vi "Send Reply.vi"(8 "错误输入（无错误）":errorcluster, 9 "Data":variant, 10 "请求":T1, 11 "Send Q":refnum<queue>) -> (0 "error out":errorcluster, 3 "Send Q":refnum<queue>)   [LabVIEW 2020, in "TCP Communication.lvlib"]
uses:
  TCP Communication.lvlib
  Requset.ctl
  Reply.ctl
  Data Type.ctl
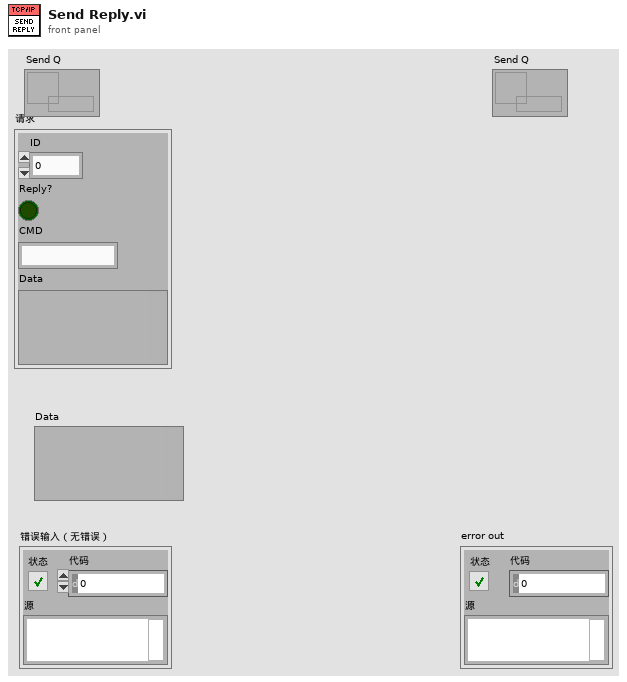
[diagram p1: front panel]
types:
  T1 = typedef "TCP Communication.lvlib/Requset.ctl" = cluster{"ID":i32, "Reply?":bool, "CMD":string, "Data":variant}
  T2 = typedef "TCP Communication.lvlib/Data Type.ctl" = enum16{"Data Stream", "Status", "Request", "Reply"}
  T3 = typedef "TCP Communication.lvlib/Reply.ctl" = cluster{"ID":i32, "CMD":string, "Data":variant}
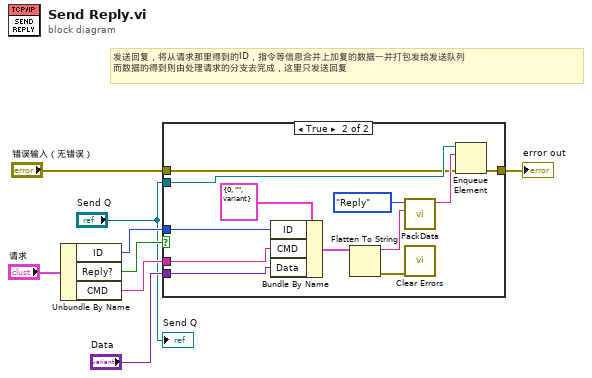
[diagram p0: block diagram]
diagram:
  # "发送回复，将从请求那里得到的ID，指令等信息合并上加复的数据一并打包发给发送队列\n而数据的得到则由处理请求的分支去完成，这里只发送回复"
  n1 = Unbundle By Name("请求") -> ("ID"=w7:i32, "Reply?"=w8:bool, "CMD"=w6:string)
  n2 = case shown="True" w8 {
    tunnel: w7 -> [_ w20]
    tunnel: w6 -> [_ w19]
    tunnel: "Send Q" -> [_ w15]
    tunnel: "Data" -> [_ w13]
    tunnel: [w9 w11] -> w3
    tunnel: "错误输入（无错误）" -> [w9 w10]
    frame False {
    }
    frame True {
      n3 = Bundle By Name(cluster=T3 {"ID"=0, "CMD"="", "Data"=variant} ("回复"), "ID"=w20, "CMD"=w19, "Data"=w13) -> (w18:T3)
      n4 = Flatten To String(anything=w18) -> (data string=w17:string, error out=w12:errorcluster)  [unwired: 3 in, 1 out]
      n5 = call "PackData.vi"("字符串输入"=w17, "Data Type"=Data_Type."Reply") -> ("字符串输出"=w14:string)  [unwired: 9 in]
      n6 = call <vilib>:"Clear Errors.vi"("error in (no error)"=w12) -> ()  [unwired: 5 in, 2 out]
      n7 = Enqueue Element(queue=w15, element=w14, error in (no error)=w10) -> (error out=w11:errorcluster)  [unwired: 1 in, 2 out]
    }
  }
  "error out" <- w3
  "Send Q" <- "Send Q"
